vi "Copy Folder and Rename Files.vi"(8 "error in (no error)":errorcluster, 9 "File Name Suffix":string, 10 "Destination Folder":path, 11 "Source Folder":path) -> (0 "error out":errorcluster)   [LabVIEW 2016, in "SLL Scripting.lvlib"]
doc: "Clear destination directory and copy the files/folders from source folder."
uses:
  SLL Scripting.lvlib
  SLL File IO/SLL File IO.lvlib
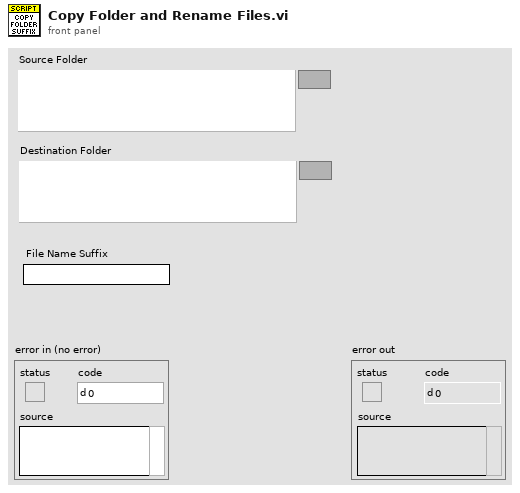
[diagram p1: front panel]
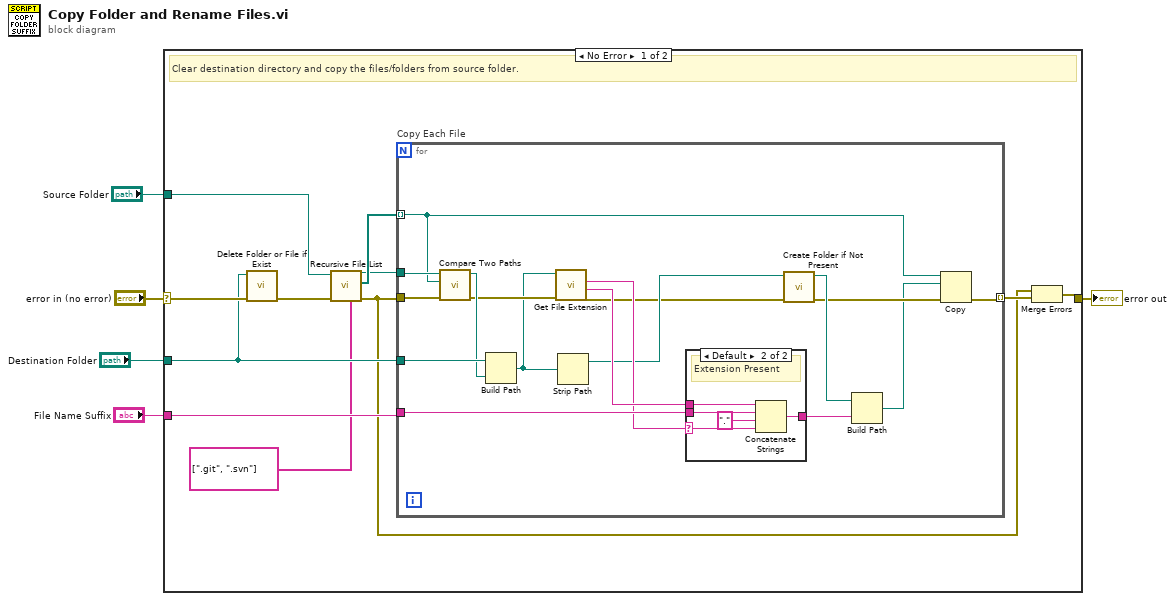
[diagram p0: block diagram]
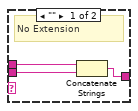
[diagram p2: hidden frame]
diagram:
  n1 = case shown="No Error" "error in (no error)" {
    selector: "error in (no error)" -> [w11 w42]
    tunnel: [w12 w42] -> w4
    tunnel: "Source Folder" -> [w15 _]
    tunnel: "Destination Folder" -> [w9 _]
    tunnel: "File Name Suffix" -> [w14 _]
    frame No Error {
      # "Clear destination directory and copy the files/folders from source folder."
      n2 = call "Delete Folder or File if Exist.vi"("error in (no error)"=w11, "Path"=w9) -> ("error out"=w10:errorcluster)  [unwired: 8 in, 1 out]
      n3 = call <vilib>:"Recursive File List.vi"("Folders to Exclude"=string[] [".git", ".svn"], "error in (no error)"=w10, "Folder Path"=w15) -> ("error out"=w6:errorcluster, "All Files in Dir"=w16:path[], "dup Folder Path"=w8:path)  [unwired: 4 in, 2 out]
      n4 = for "Copy Each File" {
        tunnel: w16 -> [w17] mode=indexing
        tunnel: w9 -> [w32]
        tunnel: w14 -> [w27]
        tunnel: w8 -> [w18]
        tunnel: w6 -> [w33]
        tunnel: [w20] -> w13 mode=indexing
        n5 = call <vilib>:"Compare Two Paths.vi"("error in (no error)"=w33, "Path 2"=w17, "Path 1"=w18) -> ("error out"=w30:errorcluster, "Relative Path from 1 to 2"=w31:path)  [unwired: 5 in, 2 out]
        n6 = Build Path(base path=w32, name or relative path=w31) -> (appended path=w29:path)
        n7 = call <vilib>:"Get File Extension.vi"("error in (no error)"=w30, "file"=w29) -> ("error out"=w24:errorcluster, "filename without extension"=w28:string, "lowercase file extension"=w26:string)  [unwired: 5 in, 2 out]
        n8 = Strip Path(path=w29) -> (stripped path=w25:path)  [unwired: 1 out]
        n9 = case shown="Default" w26 {
          selector: w26 -> [_ w38]
          tunnel: w28 -> [w36 w41]
          tunnel: w27 -> [w35 w40]
          tunnel: [w34 w37] -> w22
          frame "" {
            # "No Extension"
            n10 = Concatenate Strings(w36, w35) -> (w34:string)
          }
          frame Default {
            # "Extension Present"
            n11 = Concatenate Strings(w41, w40, "." ("string"), w38) -> (w37:string)
          }
        }
        n12 = call "Create Folder if Not Present.vi"("error in (no error)"=w24, "Path"=w25) -> ("error out"=w21:errorcluster, "Path out"=w23:path)  [unwired: 8 in]
        n13 = Build Path(base path=w23, name or relative path=w22) -> (appended path=w19:path)
        n14 = Copy(8:w21, 10:w19, 11:w17) -> (0:w20:errorcluster)  [unwired: 2 in, 2 out]
      }
      n15 = Merge Errors(w6, w13) -> (w12:errorcluster)
    }
    frame Error {
    }
  }
  "error out" <- w4
